vi "FuncVI-FileLoadSS.vi"(5 "InstanceRef":T2, 9 "arg list":T1[](array[typedef]) {"num" format="%.2f"}) -> (0 "error out":bool, 3 "result":T1 {"num" format="%.2f"})   [LabVIEW 2021]
doc: "::: CalcExpress Toolkit :::\nCopyright (c) 2000-2026 Konstantin Shifershteyn. All rights reserved."
uses:
  cetypes.llb/CalcExpress Function Argument Info.ctl
  cetypes.llb/CalcExpress Instance RefNum.ctl
panel:
  in  "max arg num":i32=5
  in  "min arg num":i32=2
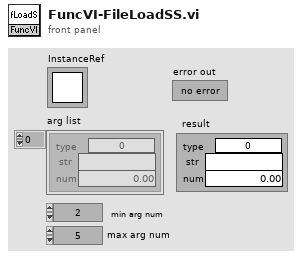
[diagram p1: front panel]
types:
  T1 = typedef "CalcExpress Function Argument Info.ctl" = cluster{"type":u32, "str":string, "num":dbl}
  T2 = typedef "CalcExpress Instance RefNum.ctl" = refnum<k1>
  T3 = cluster{"index":i32, "data type":enum32{"String", "DBL Number", "identifier", "1D Array of DBL", "2D Array of DBL", "CDB Number", "1D Array of CDB", "2D Array of CDB", "1D Array of String", "2D Array of String", "Unknown data type"}, "default num":dbl, "default str":string}[]
  T4 = enum32{"String", "DBL Number", "identifier", "1D Array of DBL", "2D Array of DBL", "CDB Number", "1D Array of CDB", "2D Array of CDB", "1D Array of String", "2D Array of String", "Unknown data type"}
  T5 = enum32{"existing file", "new file", "new or existing file", "existing dir", "new dir", "new or existing dir", "existing file (use LLBs)", "new file (use LLBs)", "new or existing file (use LLBs)", "new or existing file or directory (use LLBs)", "existing dir (use LLBs)", "new dir (use LLBs)", "new or existing dir (use LLBs)", "existing file or dir", "new file or dir", "new or existing file or dir", "existing file or dir (use LLBs)", "new file or dir (use LLBs)"}
  T6 = typedef "VarMan Variable Context Handle.ctl" = i32
  T7 = cluster{"type: use this constant to specify a predefined type code":enum32{"String", "DBL Number", "identifier", "1D Array of DBL", "2D Array of DBL", "CDB Number", "1D Array of CDB", "2D Array of CDB", "1D Array of String", "2D Array of String", "Unknown data type"}, string, dbl}
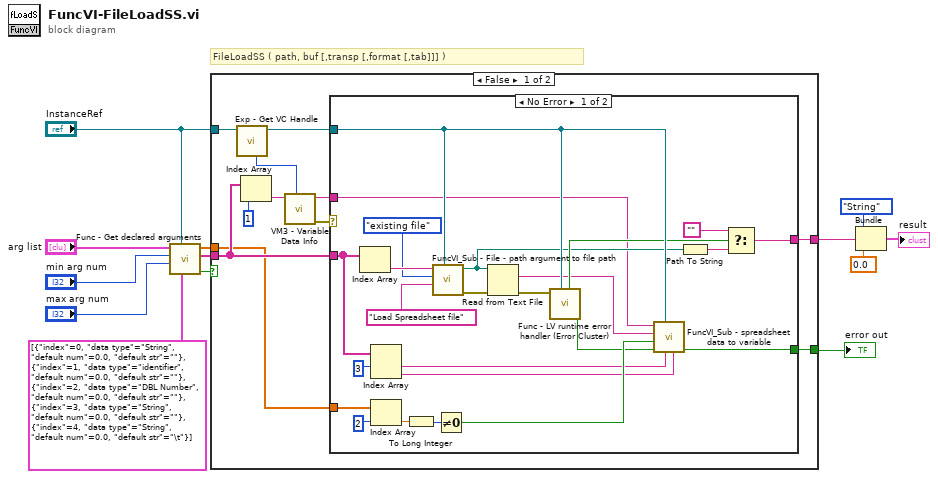
[diagram p0: block diagram]
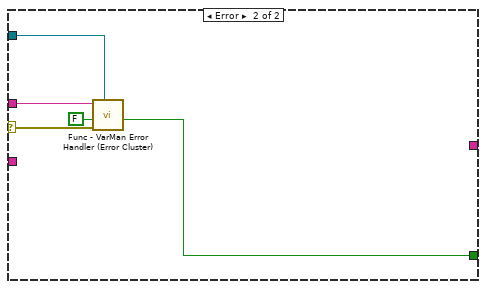
[diagram p2: hidden frame]
diagram:
  # "FileLoadSS ( path, buf [,transp [,format [,tab]]] )"
  n1 = call "Func - Get declared arguments.vi"("arg descriptors"=T3 [{"index"=0, "data type"=enum."String", "default num"=0.0, "default str"=""}, {"index"=1, "data type"=enum."identifier", "default num"=0.0, "default str"=""}, {"index"=2, "data type"=enum."DBL Number", "default num"=0.0, "default str"=""}, {"index"=3, "data type"=enum."String", "default num"=0.0, "default str"=""}, {"index"=4, "data type"=enum."String", "default num"=0.0, "default str"="\t"}] ("args descriptors"), "InstanceRef"="InstanceRef", "max arg num"="max arg num", "min arg num"="min arg num", "arg list"="arg list") -> ("error out"=w7:bool, "str list"=w8:string[], "num list"=w4:dbl[])  [unwired: 3 in, 1 out]
  n2 = case shown="False" w7 {
    selector: w7 -> [_ w54]
    tunnel: [w19 w54] -> w11
    tunnel: "InstanceRef" -> [w21 _]
    tunnel: w8 -> [w22 _]
    tunnel: [w24 _] -> w3
    tunnel: w4 -> [w18 _]
    frame False {
      n3 = call "Exp - Get VC Handle.vi"("InstanceRef"=w21) -> ("dup InstanceRef"=w20:T2, "VC Handle"=w14:T6)  [unwired: 5 in, 2 out]
      n4 = Index Array(array=w22, index=1) -> (element=w15:string)
      n5 = call "VM3 - Variable Data Info.vi"("VC Handle"=w14, "name_spec"=w15) -> ("error out"=w16:errorcluster, "dup name_spec"=w17:string)  [unwired: 4 in, 4 out]
      n6 = case shown="No Error" w16 {
        selector: w16 -> [_ w49]
        tunnel: [w34 _] -> w24
        tunnel: w22 -> [w41 _]
        tunnel: w20 -> [w33 w53]
        tunnel: [w45 w50] -> w19
        tunnel: w18 -> [w42 _]
        tunnel: w17 -> [w26 w52]
        frame No Error {
          n7 = Index Array(array=w41) -> (element=w48:string)  [unwired: 1 in]
          n8 = Index Array(array=w41, index #1=3) -> (element #1=w37:string, element #2=w25:string)  [unwired: 1 in]
          n9 = Index Array(array=w42, index=2) -> (element=w39:dbl)
          n10 = To Long Integer(number=w39) -> (32bit integer=w40:i32)
          n11 = call "FuncVI_Sub - File - path argument to file path.vi"("InstanceRef"=w33, "prompt"="Load Spreadsheet file", "select mode (2)"=T5."existing file", "arg: file path"=w48) -> ("error out"=w28:errorcluster, "file path"=w27:path)  [unwired: 5 in, 1 out]
          n12 = Not Equal To 0?(x=w40) -> (x != 0?=w38:bool)
          n13 = Read from Text File(file (use dialog)=w27, error in=w28) -> (text=w29:string, error out=w30:errorcluster)  [unwired: 2 in, 2 out]
          n14 = call "Func - LV runtime error handler (Error Cluster).vi"("InstanceRef"=w33, "LabVIEW error"=w30) -> ("error out"=w31:bool, "LV error status"=w32:bool)  [unwired: 4 in, 2 out]
          n15 = call "FuncVI_Sub - spreadsheet data to variable.vi"("delimiter (Tab)"=w25, "format string"=w37, "CE InstanceRef"=w33, "error in"=w31, "transpose"=w38, "spreadsheet string"=w29, "var name"=w26) -> ("error out"=w45:bool)  [unwired: 4 in]
          n16 = Path To String(path=w27) -> (string=w36:string)
          n17 = Select(t="", s=w32, f=w36) -> (s? t:f=w34:string)
        }
        frame Error {
          n18 = call "Func - VarMan Error Handler (Error Cluster).vi"("InstanceRef"=w53, "VarMan VI error in"=w49, "error status before"=FALSE, "var name"=w52) -> ("FuncVI error out"=w50:bool)  [unwired: 5 in, 2 out]
        }
      }
    }
    frame True {
    }
  }
  "error out" <- w11
  n19 = Bundle("type: use this constant to specify a predefined type code"=T4."String", w3, 0.0) -> (→"result":T7)  [unwired: 1 in]
